vi "Read Registry.vi"(8 "error in (no error)":errorcluster) -> (0 "error out":errorcluster, 1 "Key":string, 2 "ID":string, 3 "Date":timestamp)   [LabVIEW 2020, in "Data Viewer.lvlib"]
uses:
  Data Viewer.lvlib
  <vilib>/registry/registry.llb/Registry RtKey.ctl
  <vilib>/registry/registry.llb/Registry SAM.ctl
  <vilib>/registry/registry.llb/Write Registry Value Simple STR.vi
  <vilib>/registry/registry.llb/Read Registry Value Simple STR.vi
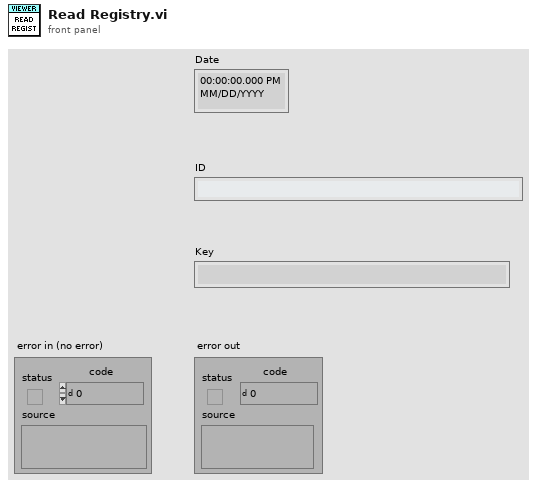
[diagram p1: front panel]
types:
  T1 = typedef "Registry SAM.ctl" = enum32{"KEY_QUERY_VALUE", "KEY_SET_VALUE", "KEY_CREATE_SUB_KEY", "KEY_ENUMERATE_SUB_KEYS", "KEY_NOTIFY", "KEY_CREATE_LINK", "KEY_READ", "KEY_WRITE", "KEY_ALL_ACCESS", "KEY_READ | KEY_WRITE"}
  T2 = typedef "Registry RtKey.ctl" = enum32{"HKEY_CLASSES_ROOT", "HKEY_CURRENT_USER", "HKEY_LOCAL_MACHINE", "HKEY_USERS", "HKEY_PERFORMANCE_DATA", "HKEY_CURRENT_CONFIG", "HKEY_DYN_DATA"}
  T3 = enum32{"Unknown", "REG_CREATED_NEW_KEY", "REG_OPENED_EXISTING_KEY"}
  T4 = typedef "Registry refnum.ctl" = refnum<k1>
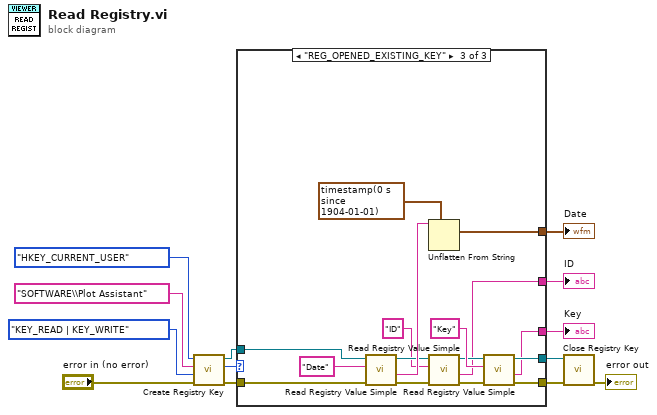
[diagram p0: block diagram]
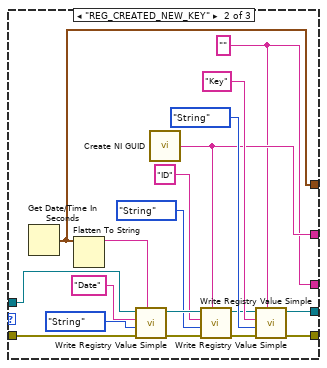
[diagram p3: hidden frame]
diagram:
  n1 = call <vilib>:"Create Registry Key.vi"("error in (no error)"="error in (no error)", "security access mask (KEY_READ | KEY_WRITE)"=Registry_SAM."KEY_READ | KEY_WRITE", "subkey"="SOFTWARE\\Plot Assistant", "root key (HKEY_LOCAL_MACHINE)"=Registry_RtKey."HKEY_CURRENT_USER") -> ("error out"=w8:errorcluster, "action taken"=w10:T3, "refnum out"=w9:T4)  [unwired: 5 in]
  n2 = case shown="\"REG_OPENED_EXISTING_KEY\"" w10 {
    tunnel: w9 -> [w15 w33 w49]
    tunnel: w8 -> [w14 w30 w47]
    tunnel: [w15 w20 w37] -> w7
    tunnel: [w14 w19 w36] -> w6
    tunnel: [_ w18 w44] -> w4
    tunnel: [_ w17 w34] -> w3
    tunnel: [_ w16 w35] -> w2
    frame "Unknown", Default {
    }
    frame "REG_CREATED_NEW_KEY" {
      w16 = "" ("String/Binary data")
      n3 = Get Date/Time In Seconds() -> (seconds since 1Jan1904=w18:timestamp)
      n4 = Flatten To String(anything=w18) -> (data string=w29:string)  [unwired: 3 in, 2 out]
      n5 = call-poly <vilib>:"Write Registry Value Simple.vi"("String/Binary data"=w29, "error in (no error)"=w30, "simple data type"=enum16{"String", "Binary", "DWORD"}."String", "value"="Date", "refnum"=w33) -> ("error out"=w27:errorcluster, "refnum out"=w28:T4)  [unwired: 3 in]
      n6 = call <vilib>:"Create NI GUID.vi"() -> ("NI GUID"=w17:string)
      n7 = call-poly <vilib>:"Write Registry Value Simple.vi"("String/Binary data"=w17, "error in (no error)"=w27, "simple data type"=enum16{"String", "Binary", "DWORD"}."String", "value"="ID", "refnum"=w28) -> ("error out"=w21:errorcluster, "refnum out"=w22:T4)  [unwired: 3 in]
      n8 = call-poly <vilib>:"Write Registry Value Simple.vi"("String/Binary data"=w16, "error in (no error)"=w21, "simple data type"=enum16{"String", "Binary", "DWORD"}."String", "value"="Key", "refnum"=w22) -> ("error out"=w19:errorcluster, "refnum out"=w20:T4)  [unwired: 3 in]
    }
    frame "REG_OPENED_EXISTING_KEY" {
      n9 = call-poly <vilib>:"Read Registry Value Simple.vi"("error in (no error)"=w47, "value"="Date", "refnum"=w49) -> ("error out"=w42:errorcluster, "String/Binary data"=w45:string, "refnum out"=w43:T4)  [unwired: 3 in, 1 out]
      n10 = Unflatten From String(type=timestamp(0 s since 1904-01-01) ("*(type *) &x"), binary string=w45) -> (value=w44:timestamp)  [unwired: 3 in, 2 out]
      n11 = call-poly <vilib>:"Read Registry Value Simple.vi"("error in (no error)"=w42, "value"="ID", "refnum"=w43) -> ("error out"=w38:errorcluster, "String/Binary data"=w34:string, "refnum out"=w39:T4)  [unwired: 3 in, 1 out]
      n12 = call-poly <vilib>:"Read Registry Value Simple.vi"("error in (no error)"=w38, "value"="Key", "refnum"=w39) -> ("error out"=w36:errorcluster, "String/Binary data"=w35:string, "refnum out"=w37:T4)  [unwired: 3 in, 1 out]
    }
  }
  "Date" <- w4
  "ID" <- w3
  "Key" <- w2
  n13 = call <vilib>:"Close Registry Key.vi"("error in (no error)"=w6, "refnum"=w7) -> ("error out"=→"error out":errorcluster)  [unwired: 5 in]
